vi "new_vi.vi"() -> ()   [LabVIEW 2014]
panel:
  out "vi refnum":refnum<vi>
  out "error out":errorcluster
  in  "vi type (standard vi)":T1(ring)
  in  "error in (no error)":errorcluster
  in  "options":u32
  in  "password":string
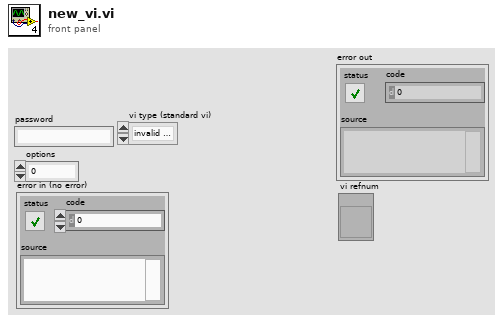
[diagram p1: front panel]
types:
  T1 = enum32{"invalid VI type", "Standard VI", "Control VI", "Global VI", "Polymorphic VI", "Configuration VI", "SubSystem", "Facade VI", "Method VI", "Statechart Diagram VI"}
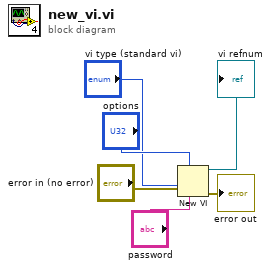
[diagram p0: block diagram]
diagram:
  n1 = New VI(6:"password", 7:"options", 8:"error in (no error)", 9:"vi type (standard vi)") -> (0:→"error out":errorcluster, 3:→"vi refnum":refnum<vi>)  [unwired: 3 in]
